vi "Image Selector.vi"(8 "Result":T1, 10 "Display ON/OFF":bool, 11 "Relative folder path name":path) -> (3 "Path to PNG file":path)   [LabVIEW 2018, in "Pass Fail Display.lvlib"]
doc: "This VI selects the right image, according to the SN Status and Display ON/OFF controls."
uses:
  Pass Fail Display.lvlib
  Result--enum.ctl
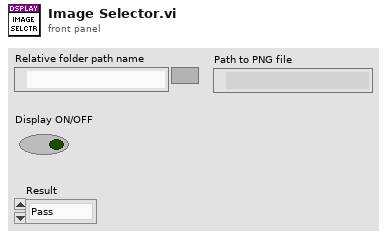
[diagram p1: front panel]
types:
  T1 = typedef "Pass Fail Display.lvlib/Result--enum.ctl" = enum16{"Pass", "Fail"}
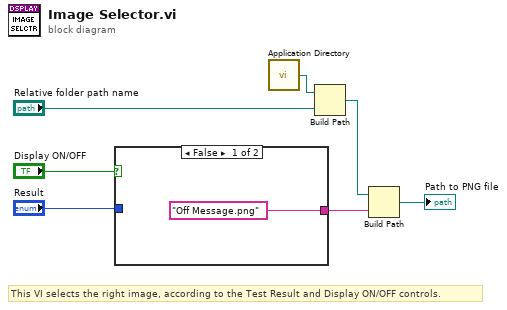
[diagram p0: block diagram]
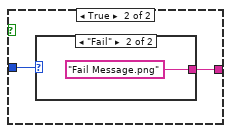
[diagram p2: hidden frame]
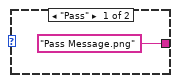
[diagram p3: hidden frame]
diagram:
  # "This VI selects the right image, according to the Test Result and Display ON/OFF controls."
  n1 = case shown="False" "Display ON/OFF" {
    tunnel: "Result" -> [_ w10]
    tunnel: ["Off Message.png" w9] -> w1
    frame False {
    }
    frame True {
      n2 = case shown="\"Fail\"" w10 {
        tunnel: ["Pass Message.png" "Fail Message.png"] -> w9
        frame "Pass" {
        }
        frame "Fail" {
        }
      }
    }
  }
  n3 = call <vilib>:"Application Directory.vi"() -> ("Application Directory"=w4:path)
  n4 = Build Path(base path=w4, name or relative path="Relative folder path name") -> (appended path=w2:path)
  n5 = Build Path(base path=w2, name or relative path=w1) -> (appended path=→"Path to PNG file":path)
